vi "Chain.vi"(10 "Order":i32, 11 "Source to Sink Array":T2) -> (3 "Node to Order-Length Paths":map{i32, map{T1, T1[][]}}(c390))   [LabVIEW 2020]
uses:
  Node.ctl
  Source to Sink Array.ctl
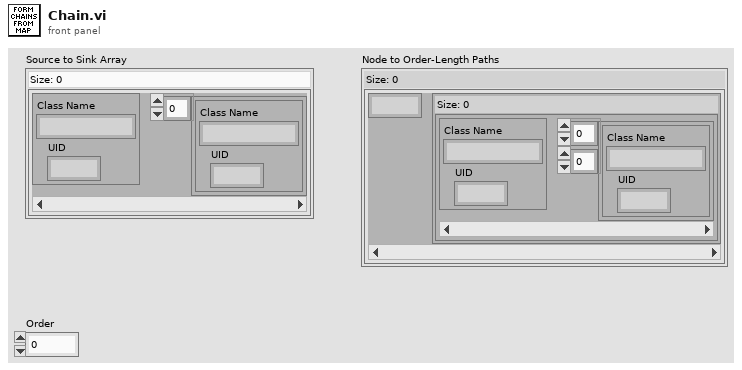
[diagram p1: front panel]
types:
  T1 = typedef "Node.ctl" = cluster{"Class Name":string, "UID":i32}
  T2 = typedef "Source to Sink Array.ctl" = map{T1, T1[]}
  T3 = map{i32, map{cluster{"Class Name":string, "UID":i32}, cluster{"Class Name":string, "UID":i32}[][]}}
  T4 = map{cluster{"Class Name":string, "UID":i32}, cluster{"Class Name":string, "UID":i32}[][]}
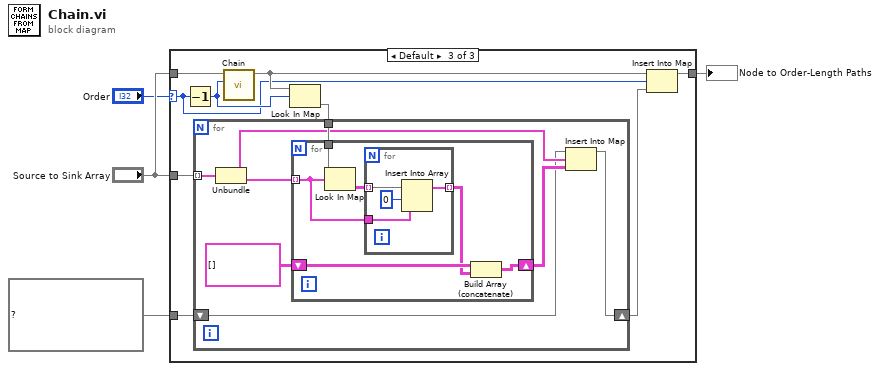
[diagram p0: block diagram]
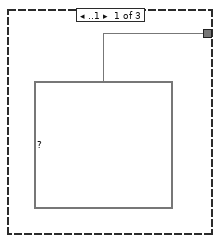
[diagram p2: hidden frame]
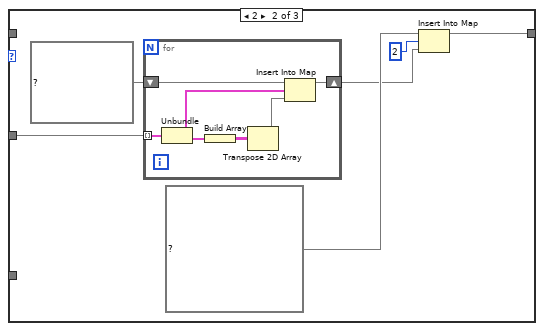
[diagram p3: hidden frame]
diagram:
  n1 = case shown="Default" "Order" {
    selector: "Order" -> [_ _ w19]
    tunnel: "Source to Sink Array" -> [_ _ w27]
    tunnel: "Source to Sink Array" -> [_ w10 w26]
    tunnel: map{T1, T1[][]} {} ("Source to Sink Array") -> [_ _ w25]
    tunnel: [T3 {} ("map") w6 w20] -> w1
    frame ..1 {
    }
    frame 2 {
      n2 = for {
        tunnel: w10 -> [w18] mode=indexing
        shift-right: [w14] -> w7
        shift-left: T4 {} ("map") -> [w17]
        n3 = Unbundle(w18) -> ("Source"=w16:T1, "Sinks"=w15:T1[])
        n4 = Build Array(w15) -> (w13:T1[][])
        n5 = Transpose 2D Array(2D array=w13) -> (transposed array=w12:T1[][])
        n6 = Insert Into Map(map in=w17, key=w16, value=w12) -> (map out=w14:T4)  [unwired: 2 out]
      }
      n7 = Insert Into Map(map in=T3 {} ("map"), key=2, value=w7) -> (map out=w6:T3)  [unwired: 2 out]
    }
    frame Default {
      n8 = Decrement(x=w19) -> (x-1=w22:i32)
      n9 = call "Chain.vi"("Order"=w22, "Source to Sink Array"=w27) -> ("Node to Order-Length Paths"=w23:map{i32, map{T1, T1[][]}})  [unwired: 9 in]
      n10 = Look In Map(map=w23, key=w22) -> (value=w24:map{T1, T1[][]})  [unwired: 1 in, 1 out]
      n11 = for {
        tunnel: w24 -> [w33]
        tunnel: w26 -> [w35] mode=indexing
        shift-right: [w29] -> w21
        shift-left: w25 -> [w30]
        n12 = Unbundle(w35) -> ("Source"=w32:T1, "Sinks"=w34:T1[])
        n13 = for {
          tunnel: w34 -> [w39] mode=indexing
          tunnel: w33 -> [w41]
          shift-right: [w37] -> w31
          shift-left: T1[][] [] ("Nodes") -> [w38]
          n14 = Look In Map(map=w41, key=w39) -> (value=w40:T1[][])  [unwired: 1 in, 1 out]
          n15 = for {
            tunnel: w40 -> [w45] mode=indexing
            tunnel: w39 -> [w43]
            tunnel: [w42] -> w36 mode=indexing
            n16 = Insert Into Array(array=w45, index=0, new element=w43) -> (w42:T1[])
          }
          n17 = Build Array (concatenate)(w38, w36) -> (w37:T1[][])
        }
        n18 = Insert Into Map(map in=w30, key=w32, value=w31) -> (map out=w29:map{T1, T1[][]})  [unwired: 2 out]
      }
      n19 = Insert Into Map(map in=w23, key=w19, value=w21) -> (map out=w20:map{i32, map{T1, T1[][]}})  [unwired: 2 out]
    }
  }
  "Node to Order-Length Paths" <- w1
